vi "1_Boolean_Adder(Training).vi"() -> ()   [LabVIEW 2020]
uses:
  <vilib>/Ngene/Deep Learning Toolkit/Toolkit/NN_Train/Controls/NN_Train_Params.ctl
  <vilib>/Ngene/Deep Learning Toolkit/Toolkit/NN_Train/Controls/NN_Train_Optimizer.ctl
  <vilib>/Ngene/Deep Learning Toolkit/Toolkit/NN_Train/Controls/NN_Train_Data_Sampling.ctl
  <vilib>/Ngene/Deep Learning Toolkit/Toolkit/NN_Train/Controls/NN_LR_Policy_Cfg.ctl
  <vilib>/Ngene/Deep Learning Toolkit/Toolkit/NN_Train/Controls/NN_LR_Policy_Type.ctl
  <vilib>/Ngene/Deep Learning Toolkit/Toolkit/NN_Train/Controls/NN_Train_Session_Data.ctl
  <vilib>/Ngene/Deep Learning Toolkit/Toolkit/NN_Data/API/DataSet/DataSet_Types/NN_DataSet(In1D_Out1D).ctl
  <vilib>/Ngene/Deep Learning Toolkit/Toolkit/NN_Data/Controls/DataRef_Types/2D/NN_Data_ref(2D_SGL).ctl
  <vilib>/Ngene/Deep Learning Toolkit/Toolkit/NN_Network/Controls/NN_Device.ctl
  <vilib>/Ngene/Deep Learning Toolkit/Toolkit/NN_Layers/Layers/FC/Controls/NN_Layer_Config(FC).ctl
  <vilib>/Ngene/Deep Learning Toolkit/Toolkit/NN_Layers/Layers/BatchNorm/Controls/NN_BN_Params.ctl
  <vilib>/Ngene/Deep Learning Toolkit/Toolkit/NN_Activations/Controls/NN_Activation_Type.ctl
  <vilib>/Ngene/Deep Learning Toolkit/Toolkit/NN_Layers/Controls/NN_Layer_Init_Params.ctl
  <vilib>/Ngene/Deep Learning Toolkit/Toolkit/NN_Layers/Controls/NN_Layer_Weight_Init_Type.ctl
  <vilib>/Ngene/Deep Learning Toolkit/Toolkit/NN_Network/Controls/NN_Save_Before_Destroy_Options.ctl
  <vilib>/Ngene/Deep Learning Toolkit/Toolkit/NN_Layers/Layers/Input/Controls/NN_Layer_Config(Input1D).ctl
  <vilib>/Ngene/Deep Learning Toolkit/Toolkit/NN_Data/Controls/NN_Data_type.ctl
  <vilib>/Ngene/Deep Learning Toolkit/Toolkit/NN_Layers/Layers/Input/NN_Layer_Create(Input1D).vi
  <vilib>/Ngene/Deep Learning Toolkit/Toolkit/NN_Layers/Layers/FC/NN_Layer_Create(FC).vi
  <vilib>/Ngene/Deep Learning Toolkit/Toolkit/NN_Train/Loss_Functions/NN_Set_Loss(MSE).vi
  <vilib>/Ngene/Deep Learning Toolkit/Toolkit/NN_Network/subVIs/NN_Predict/NN_Predict(In1D_Out1D).vi
  <vilib>/Ngene/Deep Learning Toolkit/Toolkit/Deep_Learning_Toolkit_by_Ngene.lvlib
  <vilib>/ptbypt/NI_PtbyPt.lvlib
panel:
  out "Loss Graph":cluster{"mean":dbl, "Error Rate":dbl}(graph)={"mean"=0.03092941578477621, "Error Rate"=0.0323333740234375}
  in  "stop":bool
  out "Loop Time":dbl=0.0016476999999213149 format="%#_4p"
  out "Error Rate":dbl=0.0323333740234375 format="%#_6p"
  out "Loss":sgl=0.030929416 format="%#_6p"
  in  "?":bool
  out "Session Data":T1={"Epochs"=3.788086, "Tot_Iter"=3879, "LR"=0.1, "LR_iter"=3880}
  in  "LR_Decay_Params":T2={"Policy_Type"=enum."Step", "LR0"=0.09999999999999999, "k"=10.0, "WarmUp_Policy"=enum."Ramp", "WarmUp_Iter"=1000, "WarmUp_Ratio"=1000.0} {"WarmUp_Ratio" min=1; "WarmUp_Iter" min=1; "LR0" format="%.7f"}
  in  "NN_Train_Params":T4={"Optimizer"=enum."SGD", "Beta_1"=0.9, "Beta_2"=0.9, "Weight Decay(L1)"=1e-08, "Weight Decay(L2)"=1e-08, "Data_Sampling"=enum."Random"}
  # "Overview: Demonstrates the usage of Deep Learning Toolkit for solving Boolean Adder problem.\nRequirements: DeepLTK - Deep Learning Toolkit for LabVIEW (https://www.ngene.co/deep-learning-toolkit-for-labview)\nInstructions:\n1. Run the VI.\n2. Observe how the training loss is decreasing.\n3. Observe the training speed.\n4. Press the Stop Train button when the curve stops decreasing.\nMore Examples:  https://github.com/ngenehub/deepltk_examples"
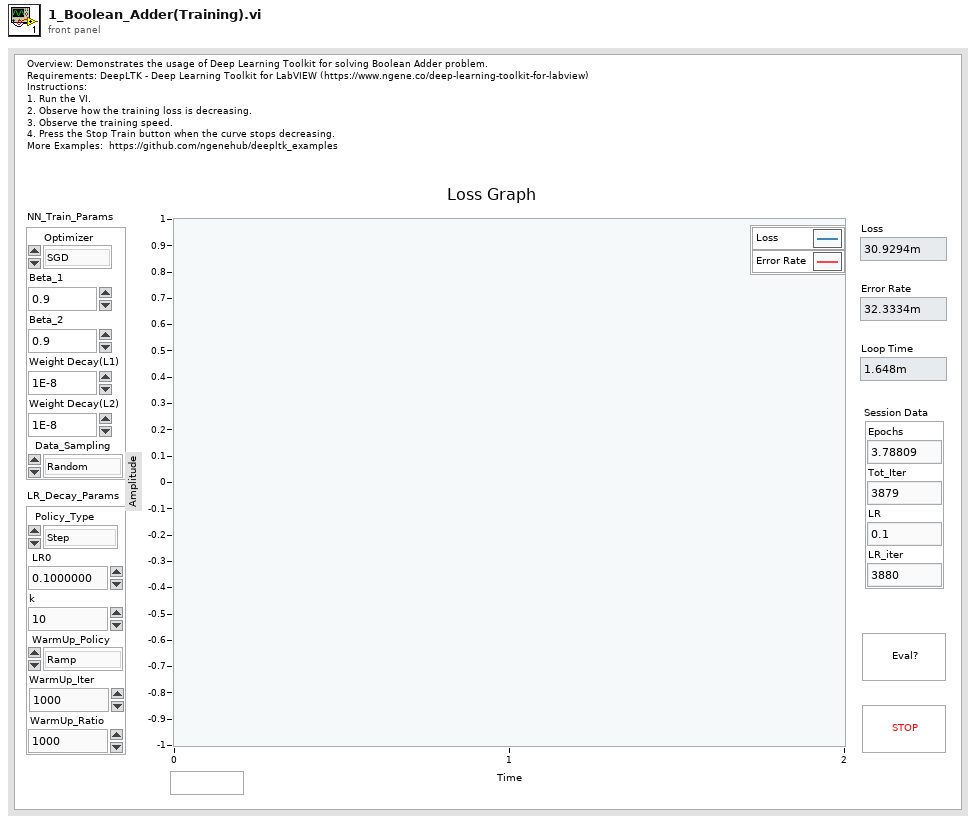
[diagram p1: front panel]
types:
  T1 = typedef "Deep_Learning_Toolkit_by_Ngene.lvlib/NN_Train_Session_Data.ctl" = cluster{"Epochs":sgl, "Tot_Iter":i32, "LR":sgl, "LR_iter":i32}
  T2 = typedef "Deep_Learning_Toolkit_by_Ngene.lvlib/NN_LR_Policy_Cfg.ctl" = cluster{"Policy_Type":T3, "LR0":dbl, "k":sgl, "WarmUp_Policy":enum16{"Step", "Ramp"}, "WarmUp_Iter":i32, "WarmUp_Ratio":sgl}
  T3 = typedef "Deep_Learning_Toolkit_by_Ngene.lvlib/NN_LR_Policy_Type.ctl" = enum16{"Manual", "Step", "Exp", "1/t"}
  T4 = typedef "Deep_Learning_Toolkit_by_Ngene.lvlib/NN_Train_Params.ctl" = cluster{"Optimizer":T5, "Beta_1":sgl, "Beta_2":sgl, "Weight Decay(L1)":sgl, "Weight Decay(L2)":sgl, "Data_Sampling":T6}
  T5 = typedef "Deep_Learning_Toolkit_by_Ngene.lvlib/NN_Train_Optimizer.ctl" = enum16{"SGD", "Adam", "Adagrad", "Adadelta", "RMSProp", "Nesterov"}
  T6 = typedef "Deep_Learning_Toolkit_by_Ngene.lvlib/NN_Train_Data_Sampling.ctl" = enum16{"Random", "Sequential"}
  T7 = typedef "Deep_Learning_Toolkit_by_Ngene.lvlib/NN_DataSet(In1D_Out1D).ctl" = cluster{"Inputs Ref.":variant, "Outputs Ref.":T8, "Dims_In":i32, "Dataset_Size":i32, "Dims_Out":i32, "Labels":string[], "File Paths":path[], "Custom_Data":variant}
  T8 = typedef "Deep_Learning_Toolkit_by_Ngene.lvlib/NN_Data_ref(2D_SGL).ctl" = refnum<data-value>
  T9 = typedef "Deep_Learning_Toolkit_by_Ngene.lvlib/NN_Layer_Config(FC).ctl" = cluster{"Name":string, "Size":i32, "BN":bool, "BN_Params":T10, "Activation":T11, "Has Bias?":bool, "Init_Params":T12, "Custom_Params":string}
  T10 = typedef "Deep_Learning_Toolkit_by_Ngene.lvlib/NN_BN_Params.ctl" = cluster{"epsilon":sgl, "momentum":sgl}
  T11 = typedef "Deep_Learning_Toolkit_by_Ngene.lvlib/NN_Activation_Type.ctl" = enum16{"Sigmoid", "ReLU", "LReLU", "ReLU6", "GELU", "tanh", "Swish", "Mish", "None"}
  T12 = typedef "Deep_Learning_Toolkit_by_Ngene.lvlib/NN_Layer_Init_Params.ctl" = cluster{"Init_Type":T13, "Value":sgl}
  T13 = typedef "Deep_Learning_Toolkit_by_Ngene.lvlib/NN_Layer_Weight_Init_Type.ctl" = enum16{"Const", "Uniform", "Gaussian", "Xavier"}
  T14 = typedef "Deep_Learning_Toolkit_by_Ngene.lvlib/NN_Device.ctl" = enum16{"CPU", "GPU"}
  T15 = typedef "Deep_Learning_Toolkit_by_Ngene.lvlib/NN_Save_Before_Destroy_Options.ctl" = cluster{"CFG?":bool, "Weights?":bool, "Render?":bool}
  T16 = typedef "Deep_Learning_Toolkit_by_Ngene.lvlib/NN_Layer_Config(Input1D).ctl" = cluster{"Name":string, "Size":i32, "Data_Type":T17, "Shift":sgl, "Scale":sgl}
  T17 = typedef "Deep_Learning_Toolkit_by_Ngene.lvlib/NN_Data_type.ctl" = enum16{"I8", "U8", "I16", "U16", "U32 ARGB", "SGL"}
  T18 = typedef "Deep_Learning_Toolkit_by_Ngene.lvlib/NN.ctl" = cluster{"Name":string, "No of Layers":i32, "mBatch":i32, "Layers":T19[], "Dimty":T20, "Dims_In":T21, "Dims_Out":T21, "Working_Dir":path, "Train?":bool, "Train_Params":T4, "LR_Update_Policy":T2, "Session Data":T1, "Ground_truth":T22, "NNg_hdls":T23, "NN_Device":T14, "GPU Id":i32, "Labels":string[], "Loss_Type":T24, "Loss_Cfg_Prms":variant, "NNG_WS":T25, "DryRun?":bool}
  T19 = typedef "Deep_Learning_Toolkit_by_Ngene.lvlib/NN_Layer_ref.ctl" = refnum<file>
  T20 = typedef "Deep_Learning_Toolkit_by_Ngene.lvlib/NN_In_Out_Dim-ty.ctl" = enum8{"In1D_Out1D", "In3D_Out1D", "In3D_Out3D", "In3D_OutBBox"}
  T21 = typedef "Deep_Learning_Toolkit_by_Ngene.lvlib/NN_Dims(C,H,W).ctl" = cluster{"C":i32, "H":i32, "W":i32}
  T22 = typedef "Deep_Learning_Toolkit_by_Ngene.lvlib/NN_Ground_truth.ctl" = cluster{"Y":variant}
  T23 = typedef "Deep_Learning_Toolkit_by_Ngene.lvlib/nng_cuda_handles.ctl" = cluster{"cudnn":u64, "cublas":u64, "stream":u64, "curand":u64}
  T24 = typedef "Deep_Learning_Toolkit_by_Ngene.lvlib/NN_Loss_Type.ctl" = enum16{"None", "MSE", "CrossEntropy", "YOLO_v2", "YOLO_v4"}
  T25 = typedef "Deep_Learning_Toolkit_by_Ngene.lvlib/NNG_WS.ctl" = cluster{"NNG_WS_Mem":T26, "Max_WS_Size":i64}
  T26 = typedef "Deep_Learning_Toolkit_by_Ngene.lvlib/NNg_WS_Mem_DVR.ctl" = refnum<data-value>
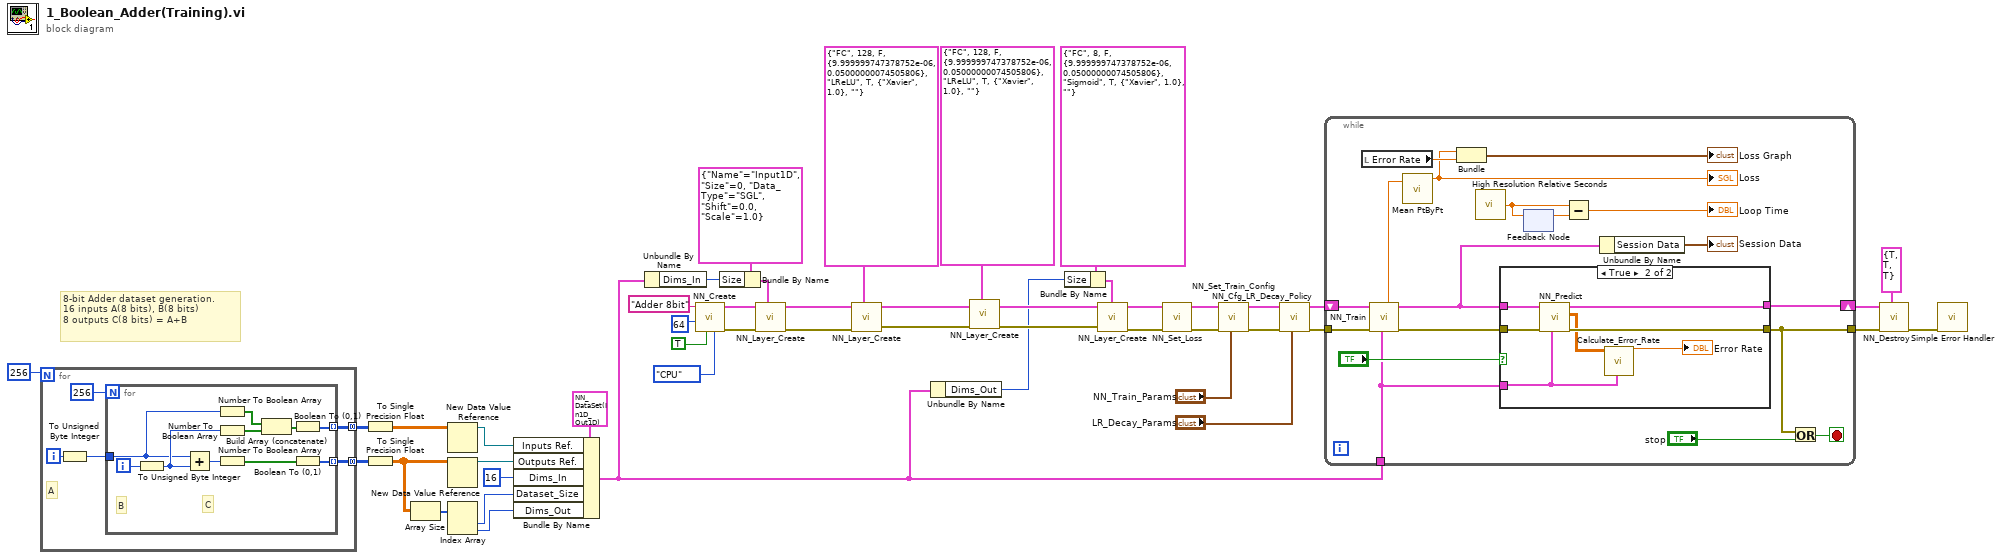
[diagram p0: block diagram]
diagram:
  # "8-bit Adder dataset generation.\n16 inputs A(8 bits), B(8 bits)\n8 outputs C(8 bits) = A+B"
  n1 = for {
    N: 256 -> [_]
    tunnel: [w51] -> w15 mode=concatenating
    tunnel: [w50] -> w14 mode=concatenating
    i -> [w49]
    # "A"
    n2 = To Unsigned Byte Integer(number=w49) -> (unsigned 8bit integer=w48:u8)
    n3 = for {
      N: 256 -> [_]
      tunnel: [w61] -> w50 mode=indexing
      tunnel: [w58] -> w51 mode=indexing
      tunnel: w48 -> [w55]
      i -> [w57]
      # "C"
      # "B"
      n4 = To Unsigned Byte Integer(number=w57) -> (unsigned 8bit integer=w56:u8)
      n5 = Add(x=w55, y=w56) -> (x+y=w59:u8)
      n6 = Number To Boolean Array(number=w55) -> (Boolean array=w53:bool[])
      n7 = Number To Boolean Array(number=w56) -> (Boolean array=w62:bool[])
      n8 = Number To Boolean Array(number=w59) -> (Boolean array=w60:bool[])
      n9 = Build Array (concatenate)(w53, w62) -> (w54:bool[])
      n10 = Boolean To (0,1)(Boolean=w54) -> (0, 1=w61:i16[])
      n11 = Boolean To (0,1)(Boolean=w60) -> (0, 1=w58:i16[])
    }
  }
  n12 = To Single Precision Float(number=w14) -> (single precision float=w8:sgl[][])
  n13 = To Single Precision Float(number=w15) -> (single precision float=w12:sgl[][])
  n14 = Array Size(array=w12) -> (size(s)=w11:i32[])
  n15 = New Data Value Reference(data value=w8) -> (data value reference=w17:refnum<data-value>)  [unwired: 1 in, 1 out]
  n16 = New Data Value Reference(data value=w12) -> (data value reference=w16:refnum<data-value>)  [unwired: 1 in, 1 out]
  n17 = Index Array(array=w11) -> (element #1=w10:i32, element #2=w9:i32)  [unwired: 2 in]
  n18 = Bundle By Name(cluster=T7 {"Inputs Ref."=variant(refnum<data-value> refnum), "Outputs Ref."=refnum, "Dims_In"=0, "Dataset_Size"=0, "Dims_Out"=0, "Labels"=[], "File Paths"=[], "Custom_Data"=variant} ("Dataset(In1D_Out1D)"), "Inputs Ref."=w17, "Outputs Ref."=w16, "Dims_In"=16, "Dataset_Size"=w10, "Dims_Out"=w9) -> (w2:T7)
  n19 = Unbundle By Name(w2) -> ("Dims_In"=w3:i32)
  n20 = call <vilib>:"NN_Create.vi"("NN_Device"=NN_Device."CPU", "Train? (false)"=TRUE, "mBatch (1)"=64, "Name"="Adder 8bit") -> ("error out"=w44:errorcluster, "NN out"=w45:T18)  [unwired: 6 in]
  n21 = Bundle By Name(cluster=T16 {"Name"="Input1D", "Size"=0, "Data_Type"=enum."SGL", "Shift"=0.0, "Scale"=1.0} ("Input1D_Cfg"), "Size"=w3) -> (w39:T16)
  n22 = call-poly <vilib>:"NN_Layer_Create.vi"("Input1D_Cfg"=w39, "error in (no error)"=w44, "NN in"=w45) -> ("error out"=w47:errorcluster, "NN out"=w46:T18)  [unwired: 6 in, 1 out]
  n23 = call-poly <vilib>:"NN_Layer_Create.vi"("FC_Cfg"=T9 {"Name"="FC", "Size"=128, "BN"=FALSE, "BN_Params"={"epsilon"=1e-05, "momentum"=0.05}, "Activation"=enum."LReLU", "Has Bias?"=TRUE, "Init_Params"={"Init_Type"=enum."Xavier", "Value"=1.0}, "Custom_Params"=""}, "error in (no error)"=w47, "NN in"=w46) -> ("error out"=w21:errorcluster, "NN out"=w22:T18)  [unwired: 6 in, 1 out]
  n24 = Unbundle By Name(w2) -> ("Dims_Out"=w4:i32)
  n25 = call-poly <vilib>:"NN_Layer_Create.vi"("FC_Cfg"=T9 {"Name"="FC", "Size"=128, "BN"=FALSE, "BN_Params"={"epsilon"=1e-05, "momentum"=0.05}, "Activation"=enum."LReLU", "Has Bias?"=TRUE, "Init_Params"={"Init_Type"=enum."Xavier", "Value"=1.0}, "Custom_Params"=""}, "error in (no error)"=w21, "NN in"=w22) -> ("error out"=w20:errorcluster, "NN out"=w19:T18)  [unwired: 6 in, 1 out]
  n26 = Bundle By Name(cluster=T9 {"Name"="FC", "Size"=8, "BN"=FALSE, "BN_Params"={"epsilon"=1e-05, "momentum"=0.05}, "Activation"=enum."Sigmoid", "Has Bias?"=TRUE, "Init_Params"={"Init_Type"=enum."Xavier", "Value"=1.0}, "Custom_Params"=""} ("FC_Cfg"), "Size"=w4) -> (w5:T9)
  n27 = call-poly <vilib>:"NN_Layer_Create.vi"("FC_Cfg"=w5, "error in (no error)"=w20, "NN in"=w19) -> ("error out"=w25:errorcluster, "NN out"=w24:T18)  [unwired: 6 in, 1 out]
  n28 = call-poly <vilib>:"NN_Set_Loss.vi"("error in (no error)"=w25, "NN in"=w24) -> ("error out"=w26:errorcluster, "NN out"=w27:T18)  [unwired: 8 in]
  n29 = call <vilib>:"NN_Set_Train_Config.vi"("NN_Train_Params"="NN_Train_Params", "error in (no error)"=w26, "NN in"=w27) -> ("error out"=w32:errorcluster, "NN out"=w37:T18)  [unwired: 7 in]
  n30 = call <vilib>:"NN_Cfg_LR_Decay_Policy.vi"("LR_Decay_Params"="LR_Decay_Params", "error in (no error)"=w32, "NN in"=w37) -> ("error out"=w31:errorcluster, "NN out"=w33:T18)  [unwired: 7 in]
  n31 = while {
    tunnel: w31 -> [w79]
    tunnel: w2 -> [w71]
    shift-right: [w75] -> w35
    shift-left: w33 -> [w80]
    tunnel: [w70] -> w34
    stop <- w65 stop-if-true
    n32 = local read "Error Rate"() -> (w72:dbl)
    n33 = call <vilib>:"NN_Train.vi"("Train Dataset"=w71, "error in (no error)"=w79, "NN in"=w80) -> ("error out"=w74:errorcluster, "NN out"=w77:T18, "Loss"=w78:sgl)  [unwired: 3 in, 3 out]
    n34 = call <vilib>:"Mean PtByPt.vi"("x"=w78) -> ("mean"=w69:dbl)  [unwired: 3 in, 1 out]
    "Loss" <- w69
    n35 = Bundle("mean"=w69, "Error Rate"=w72) -> (→"Loss Graph":cluster{"mean":dbl, "Error Rate":dbl})  [unwired: 1 in]
    n36 = call <vilib>:"High Resolution Relative Seconds.vi"() -> ("relative seconds"=w67:dbl)
    n37 = case shown="True" "?" {
      tunnel: w77 -> [w82 w87]
      tunnel: [w82 w89] -> w75
      tunnel: w74 -> [w81 w86]
      tunnel: [w81 w88] -> w70
      tunnel: w71 -> [_ w83]
      frame False {
      }
      frame True {
        n38 = call-poly <vilib>:"NN_Predict.vi"("Dataset"=w83, "error in (no error)"=w86, "NN in"=w87) -> ("error out"=w88:errorcluster, "Predictions"=w85:sgl[][], "NN out"=w89:T18)  [unwired: 6 in]
        n39 = call "Calculate_Error_Rate.vi"("Dataset(In1D_Out1D)"=w83, "Predictions"=w85) -> ("Error Rate"=→"Error Rate":dbl)  [unwired: 9 in]
      }
    }
    n40 = feedback #1() -> (w66:dbl)  [unwired: 1 in]
    n41 = feedback-in #1(w67) -> ()
    n42 = Subtract(x=w67, y=w66) -> (x-y=→"Loop Time":dbl)
    n43 = Unbundle By Name(w77) -> ("Session Data"=→"Session Data":T1)
    n44 = Or(x=w70, y="stop") -> (x .or. y?=w65:bool)
  }
  n45 = call <vilib>:"NN_Destroy.vi"("Save (T, T, T)"=T15 {"CFG?"=TRUE, "Weights?"=TRUE, "Render?"=TRUE}, "error in (no error)"=w34, "NN in"=w35) -> ("error out"=w1:errorcluster)  [unwired: 7 in, 1 out]
  n46 = call <vilib>:"Simple Error Handler.vi"("error in (no error)"=w1) -> ()  [unwired: 4 in, 5 out]
